vi "DiffDriveTrainSim_New_Mass_MOI.vi"(5 "j_KgM2":dbl=1.0, 6 "MeasurementStdDev":T1=[[0.0], [0.0], [0.0], [0.0], [0.0], [0.0], [0.0]], 7 "Mass_Kg":dbl, 8 "WheelRadius_M":dbl, 9 "TrackWidth_M":dbl, 10 "Gearing":dbl=1.0, 11 "DriveMotor":T2 {"Jr_KgM2" format="%13.5p"; "L_H" format="%13.5p"; "Kt_NMPerAmp" format="%13.5p"; "KvINV_RadPerSecPerVolt" format="%13.5p"; "R_Ohms" format="%13.5p"; "FreeSpeed_RadPerSec" format="%13.5p"; "FreeCurrent_Amps" format="%13.5p"; "StallCurrent_Amps" format="%13.5p"; "StallTorque_NM" format="%13.5p"; "nominalVoltage_Volts" format="%13.5p"}) -> (0 "Size Coerced":bool, 3 "DiffDriveTrainSim":T3 {"m_Motor"."Jr_KgM2" format="%13.5p"; "m_Motor"."L_H" format="%13.5p"; "m_Motor"."Kt_NMPerAmp" format="%13.5p"; "m_Motor"."KvINV_RadPerSecPerVolt" format="%13.5p"; "m_Motor"."R_Ohms" format="%13.5p"; "m_Motor"."FreeSpeed_RadPerSec" format="%13.5p"; "m_Motor"."FreeCurrent_Amps" format="%13.5p"; "m_Motor"."StallCurrent_Amps" format="%13.5p"; "m_Motor"."StallTorque_NM" format="%13.5p"; "m_Motor"."nominalVoltage_Volts" format="%13.5p"})   [LabVIEW 2019, in "Trajectory_Library.lvlib"]
doc: "Create a SimDrivetrain.\n\nThis class simulates the state of the drivetrain. In simulationPeriodic, users should first set inputs from motors with setInputs(double, double)}, call update(double)} to update the simulation, and set estimated encoder and gyro positions, as well as estimated odometry pose. \n \nOur state-space system is:\n \n x = [[x, y, theta, vel_l, vel_r, dist_l, dist_r]]? \n\n in the field coordinate system (dist_* are wheel distances.)\n \n u = [[voltage_l, voltage_r]]? \n\n This is typically the control input of the last timestep\n from a LTVDiffDriveController.\n \n y = x\n \n\nInputs:\n - DiffDriveTraimSim -- Data cluster\n - driveMotor -- A DCMotor representing the left side of the drivetrain.\n - gearing -- The gearing ratio between motor and wheel, as output over input. This must be the same ratio as the ratio used to identify or create the drivetrainPlant.\n - jKgMetersSquared -- The moment of inertia of the drivetrain about its center.\n - massKg -- The mass of the drivebase.\n - wheelRadiusMeters -- The radius of the wheels on the drivetrain.\n - trackWidthMeters -- The robot's track width, or distance between left and right wheels.\n - measurementStdDevs -- Standard deviations for measurements, in the form [x, y, heading, left velocity, right velocity, left distance, right distance]?. Can be null if no noise is desired. Gyro standard deviations of 0.0001 radians, velocity standard deviations of 0.05 m/s, and position measurement standard deviations of 0.005 meters are a reasonable starting point.\n\nOutputs:\n - OutDiffDriveTraimSim -- Updated data cluster.\n - Size Coerced -- If TRUE, an error occured. Execution may continue."
uses:
  Trajectory_Library.lvlib
  TypeDef/LINEAR_SYSTEM.ctl
  <vilib>/Analysis/Matrix/Datatypes/RealMatrix.ctl
  <vilib>/Analysis/Matrix/NI_Matrix.lvlib
  TypeDef/DCMOTOR.CTL
  TypeDef/DIFF_DRIVE_TRAIN_SIM.ctl
panel:
  # "<7, 1>"
  # "<States, 1>"
  # "<Outputs, 1>"
  # "<Inputs, 1>"
  # "<Outputs, 1>"
  # "<States,States>"
  # "<States,Inputs>"
  # "<Outputs,States>"
  # "<Outputs,Inputs>"
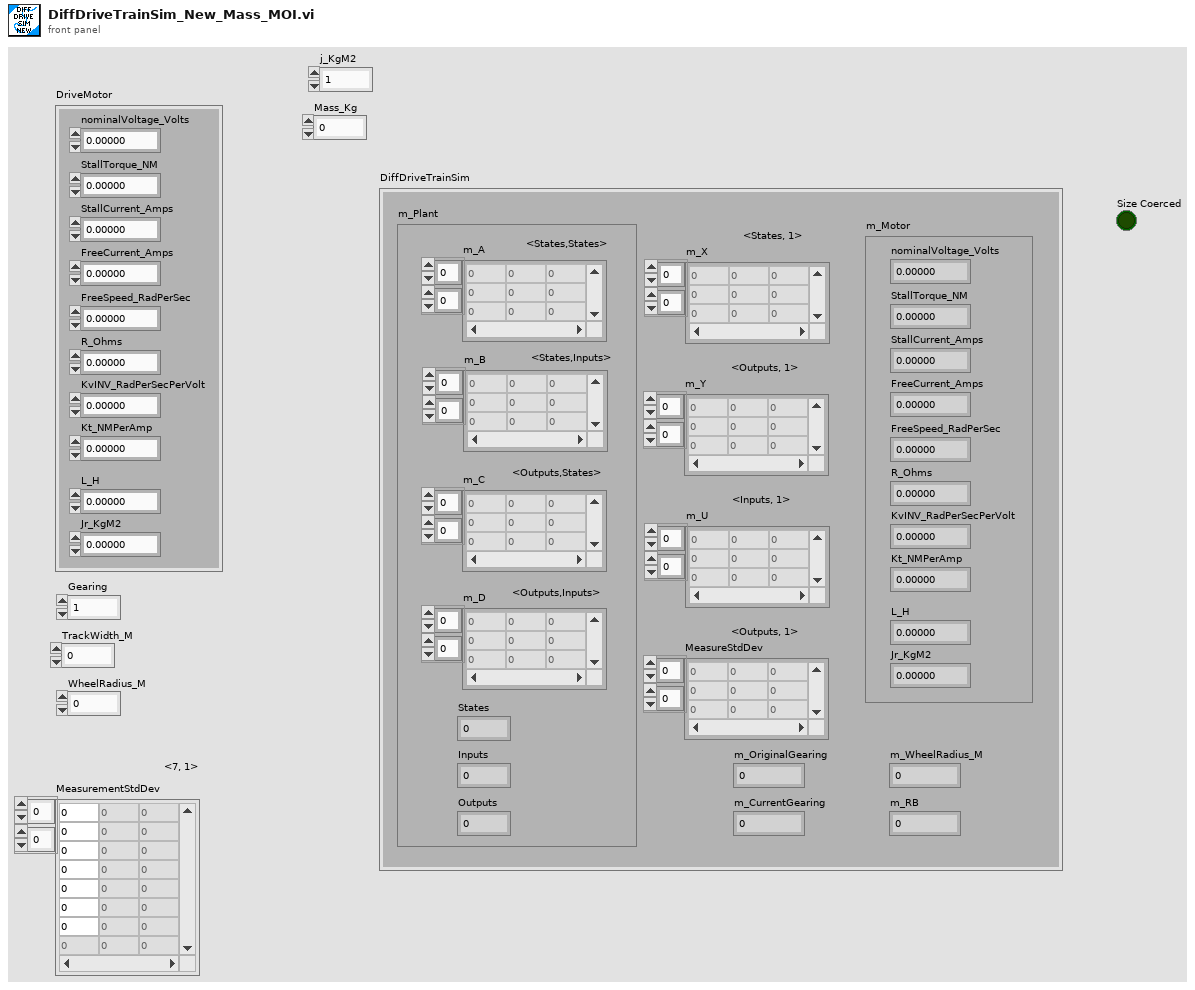
[diagram p1: front panel]
types:
  T1 = typedef "NI_Matrix.lvlib/RealMatrix.ctl" = dbl[][]
  T2 = typedef "Trajectory_Library.lvlib/DCMOTOR.CTL" = cluster{"nominalVoltage_Volts":dbl, "StallTorque_NM":dbl, "StallCurrent_Amps":dbl, "FreeCurrent_Amps":dbl, "FreeSpeed_RadPerSec":dbl, "R_Ohms":dbl, "KvINV_RadPerSecPerVolt":dbl, "Kt_NMPerAmp":dbl, "L_H":dbl, "Jr_KgM2":dbl}
  T3 = typedef "Trajectory_Library.lvlib/DIFF_DRIVE_TRAIN_SIM.ctl" = cluster{"m_Plant":T4, "m_X":T1, "m_Y":T1, "m_U":T1, "MeasureStdDev":T1, "m_Motor":T2, "m_OriginalGearing":dbl, "m_CurrentGearing":dbl, "m_WheelRadius_M":dbl, "m_RB":dbl}
  T4 = typedef "Trajectory_Library.lvlib/LINEAR_SYSTEM.ctl" = cluster{"m_A":T1, "m_B":T1, "m_C":T1, "m_D":T1, "States":i32, "Inputs":i32, "Outputs":i32}
  T5 = typedef "WPILib_Math.lvlib/LINEAR_SYSTEM.ctl" = cluster{"m_A":T1, "m_B":T1, "m_C":T1, "m_D":T1, "States":i32, "Inputs":i32, "Outputs":i32}
  T6 = typedef "WPILib_Math.lvlib/DIFF_DRIVE_TRAIN_SIM.ctl" = cluster{"m_Plant":T5, "m_X":T1, "m_Y":T1, "m_U":T1, "MeasureStdDev":T1, "m_Motor":T7, "m_OriginalGearing":dbl, "m_CurrentGearing":dbl, "m_WheelRadius_M":dbl, "m_RB":dbl}
  T7 = typedef "WPILib_Math.lvlib/DCMOTOR.CTL" = cluster{"nominalVoltage_Volts":dbl, "StallTorque_NM":dbl, "StallCurrent_Amps":dbl, "FreeCurrent_Amps":dbl, "FreeSpeed_RadPerSec":dbl, "R_Ohms":dbl, "KvINV_RadPerSecPerVolt":dbl, "Kt_NMPerAmp":dbl, "L_H":dbl, "Jr_KgM2":dbl}
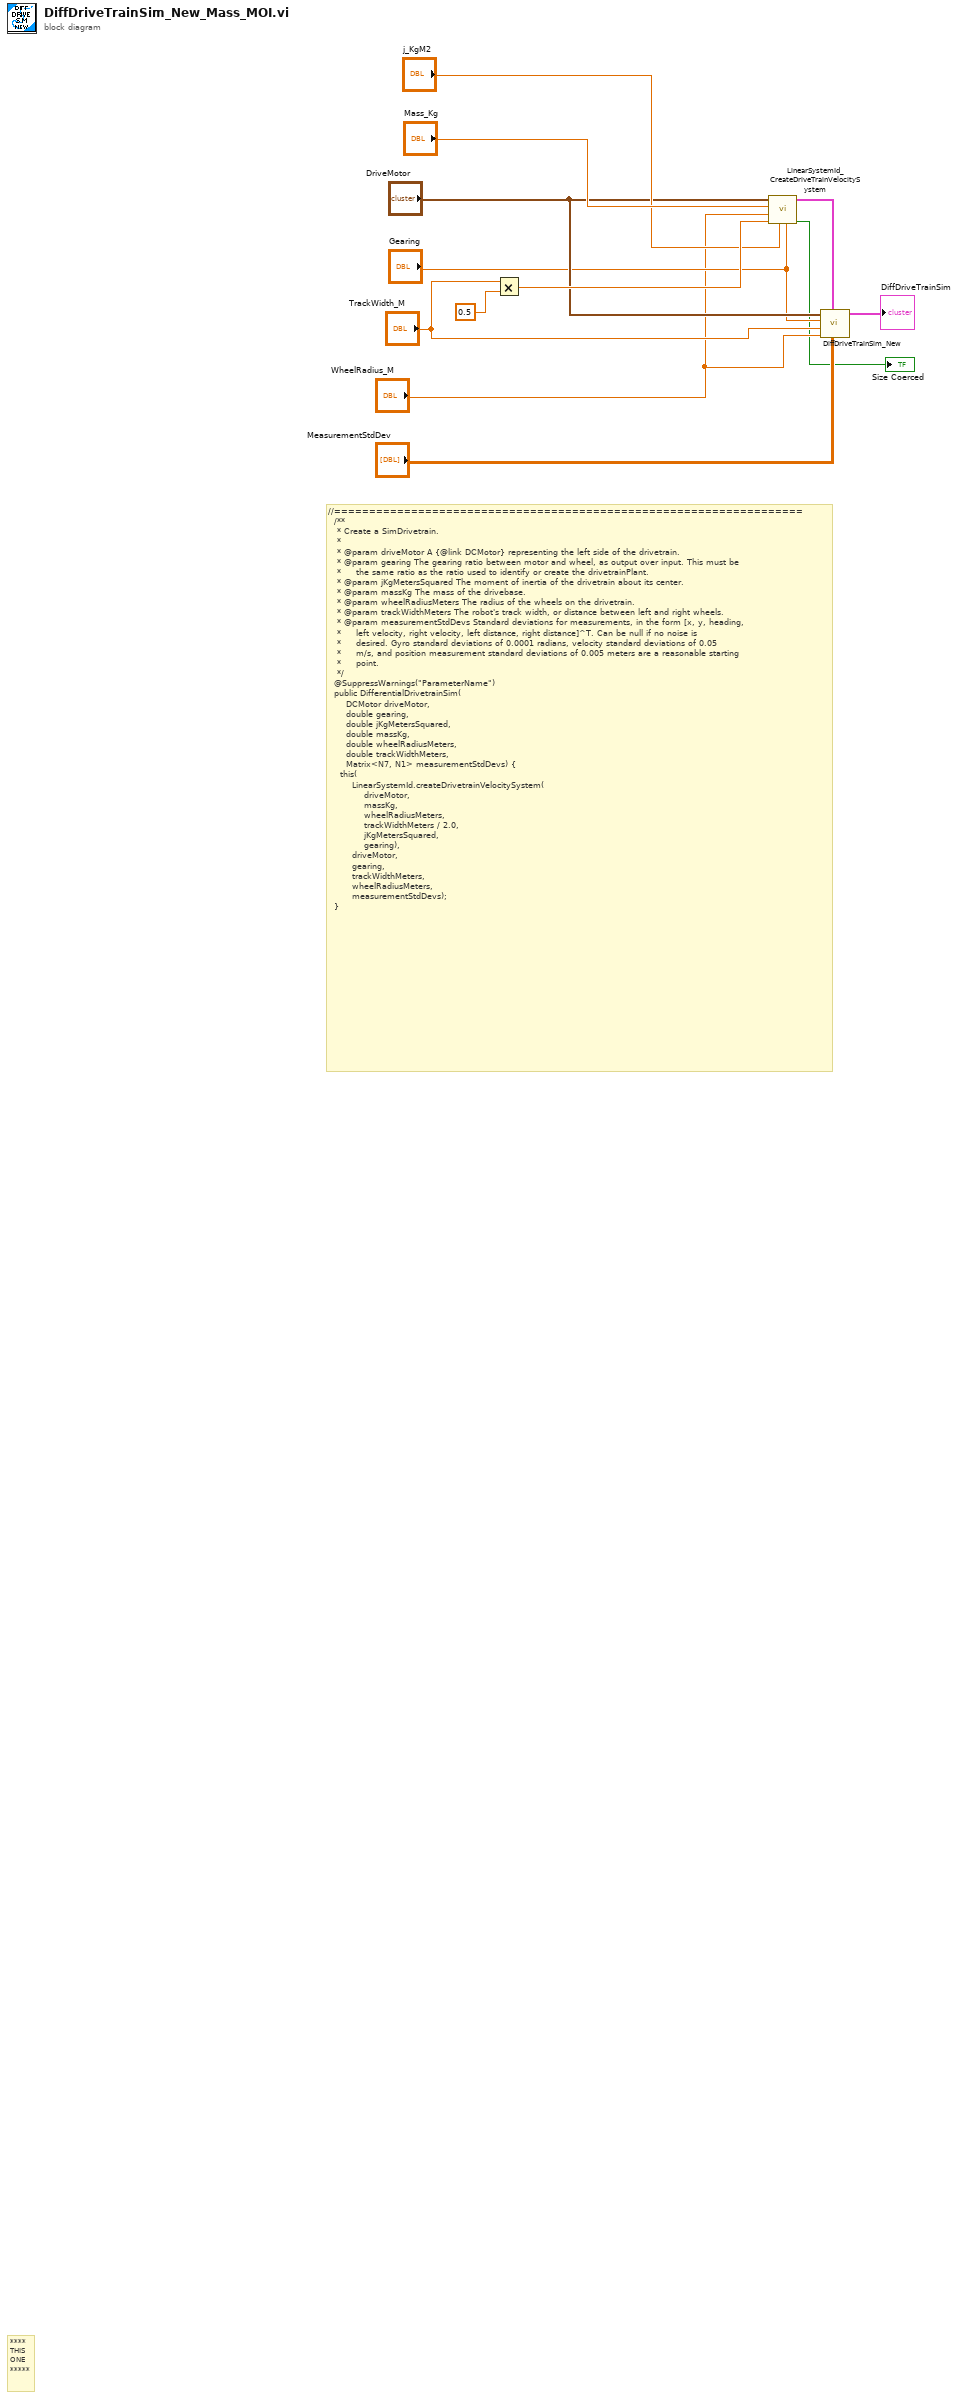
[diagram p0: block diagram]
diagram:
  # "//===================================================================\n  /**\n   * Create a SimDrivetrain.\n   *\n   * @param driveMotor A {@link DCMotor} representing the left side of the drivetrain.\n   * @param gearing The gearing ratio between motor and wheel, as output over input. This must be\n   *     the same ratio as the ratio used to identify or create the drivetrainPlant.\n   * @param jKgMetersSquared The moment of inertia of the drivetrain about its center.\n   * @param massKg The mass of the drivebase.\n   * @param wheelRadiusMeters The radius of the wheels on the drivetrain.\n   * @param trackWidthMeters The robot's track width, or distance between left and right wheels.\n   * @param measurementStdDevs Standard deviations for measurements, in the form [x, y, heading,\n   *     left velocity, right velocity, left distance, right distance]^T. Can be null if no noise is\n   *     desired. Gyro standard deviations of 0.0001 radians, velocity standard deviations of 0.05\n   *     m/s, and position measurement standard deviations of 0.005 meters are a reasonable starting\n   *     point.\n   */\n  @SuppressWarnings(\"ParameterName\")\n  public DifferentialDrivetrainSim(\n      DCMotor driveMotor,\n      double gearing,\n      double jKgMetersSquared,\n      double massKg,\n      double wheelRadiusMeters,\n      double trackWidthMeters,\n      Matrix<N7, N1> measurementStdDevs) {\n    this(\n        LinearSystemId.createDrivetrainVelocitySystem(\n            driveMotor,\n            massKg,\n            wheelRadiusMeters,\n            trackWidthMeters / 2.0,\n            jKgMetersSquared,\n            gearing),\n        driveMotor,\n        gearing,\n        trackWidthMeters,\n        wheelRadiusMeters,\n        measurementStdDevs);\n  }"
  # "****\nTHIS\nONE\n*****"
  n1 = Multiply(x="TrackWidth_M", y=0.5) -> (x*y=w9:dbl)
  n2 = call "LinearSystemId_CreateDriveTrainVelocitySystem.vi"("G"="Gearing", "JKgMetersSquared"="j_KgM2", "rbMeters"=w9, "rMeters"="WheelRadius_M", "MassKg"="Mass_Kg", "Motor"="DriveMotor") -> ("Size Coerced"=→"Size Coerced":bool, "Linearsystem"=w11:T5)  [unwired: 4 in]
  n3 = call "DiffDriveTrainSim_New.vi"("MeasurementStdDev"="MeasurementStdDev", "DriveTrainPlant"=w11, "WheelRadius_M"="WheelRadius_M", "TrackWidth_M"="TrackWidth_M", "Gearing"="Gearing", "DriveMotor"="DriveMotor") -> ("DiffDriveTrainSim"=→"DiffDriveTrainSim":T6)  [unwired: 5 in]
